vi "风速测量.vi"() -> ()   [LabVIEW 2014]
panel:
  in  "输入设备":tag="Dev2/port0/line0:2"
  in  "输出设备":tag="Dev1/port0/line0:7"
  out "测量点":u32[](array[numeric])
  out "Error Out":errorcluster caption="错误输出"
  in  "风筒直径":string
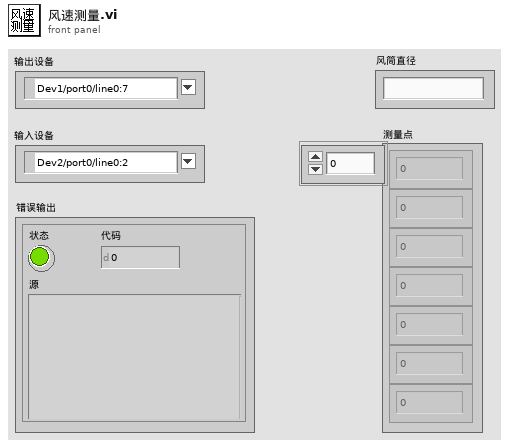
[diagram p1: front panel]
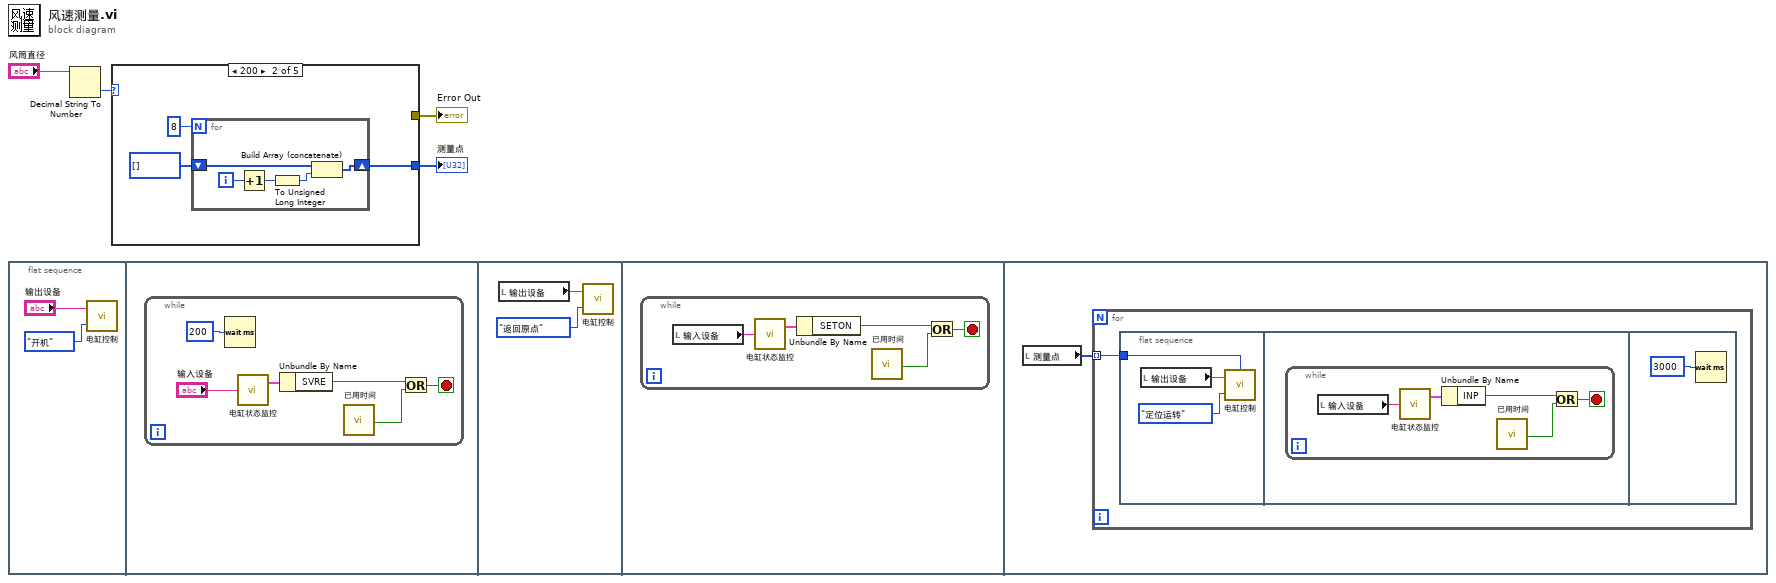
[diagram p0: block diagram]
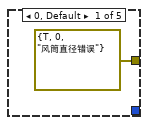
[diagram p2: hidden frame]
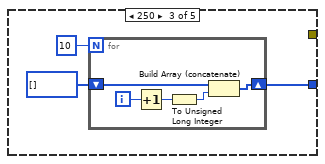
[diagram p3: hidden frame]
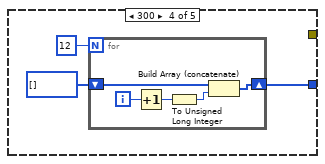
[diagram p4: hidden frame]
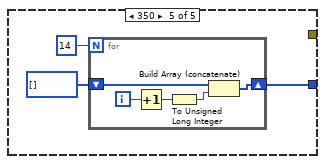
[diagram p5: hidden frame]
diagram:
  n1 = flat-sequence {
    frame #0 {
      n2 = call "电缸控制.vi"("枚举"=enum16{"开机", "返回原点", "定位运转", "报警复位"}."开机", "输出设备"="输出设备") -> ()  [unwired: 1 in, 1 out]
    }
    frame #1 {
      n3 = while {
        stop <- w9 stop-if-true
        n4 = Wait (ms)(milliseconds to wait=u32 200 ("等待时间（毫秒）")) -> ()  [unwired: 1 out]
        n5 = call "电缸状态监控.vi"("输入设备"="输入设备") -> ("电缸状态指示"=w12:cluster{"INP":bool, "SETON":bool, "SVRE":bool})  [unwired: 1 out]
        n6 = Unbundle By Name(w12) -> ("SVRE"=w11:bool)
        n7 = call "已用时间"() -> ("Time has Elapsed"=w10:bool)  [unwired: 12 in, 7 out]
        n8 = Or(x=w11, y=w10) -> (x .or. y?=w9:bool)
      }
    }
    frame #2 {
      n9 = local read "输出设备"() -> (w14:tag)
      n10 = call "电缸控制.vi"("枚举"=enum16{"开机", "返回原点", "定位运转", "报警复位"}."返回原点", "输出设备"=w14) -> ()  [unwired: 1 in, 1 out]
    }
    frame #3 {
      n11 = while {
        stop <- w15 stop-if-true
        n12 = local read "输入设备"() -> (w16:tag)
        n13 = call "电缸状态监控.vi"("输入设备"=w16) -> ("电缸状态指示"=w19:cluster{"INP":bool, "SETON":bool, "SVRE":bool})  [unwired: 1 out]
        n14 = Unbundle By Name(w19) -> ("SETON"=w18:bool)
        n15 = call "已用时间"() -> ("Time has Elapsed"=w17:bool)  [unwired: 12 in, 7 out]
        n16 = Or(x=w18, y=w17) -> (x .or. y?=w15:bool)
      }
    }
    frame #4 {
      n17 = local read "测量点"() -> (w20:u32[])
      n18 = for {
        tunnel: w20 -> [w21] mode=indexing
        n19 = flat-sequence {
          tunnel: w21 -> [w22]
          frame #0 {
            n20 = local read "输出设备"() -> (w23:tag)
            n21 = call "电缸控制.vi"("步序号"=w22, "枚举"=enum16{"开机", "返回原点", "定位运转", "报警复位"}."定位运转", "输出设备"=w23) -> ()  [unwired: 1 out]
          }
          frame #1 {
            n22 = while {
              stop <- w25 stop-if-true
              n23 = local read "输入设备"() -> (w26:tag)
              n24 = call "电缸状态监控.vi"("输入设备"=w26) -> ("电缸状态指示"=w29:cluster{"INP":bool, "SETON":bool, "SVRE":bool})  [unwired: 1 out]
              n25 = Unbundle By Name(w29) -> ("INP"=w28:bool)
              n26 = call "已用时间"() -> ("Time has Elapsed"=w27:bool)  [unwired: 12 in, 7 out]
              n27 = Or(x=w28, y=w27) -> (x .or. y?=w25:bool)
            }
          }
          frame #2 {
            n28 = Wait (ms)(milliseconds to wait=u32 3000 ("等待时间（毫秒）")) -> ()  [unwired: 1 out]
          }
        }
      }
    }
  }
  n29 = Decimal String To Number(string="风筒直径") -> (number=w3:i32)  [unwired: 2 in, 1 out]
  n30 = case shown="200" w3 {
    tunnel: [errorcluster {"status"=TRUE, "code"=0, "source"="风筒直径错误"} ("Error Out") _ _ _ _] -> w1
    tunnel: [_ w34 w40 w48 w56] -> w2
    frame 0, Default {
    }
    frame 200 {
      n31 = for {
        N: 8 -> [_]
        shift-right: [w37] -> w34
        shift-left: u32[] [] -> [w39]
        i -> [w35]
        n32 = Increment(x=w35) -> (x+1=w36:i32)
        n33 = To Unsigned Long Integer(number=w36) -> (unsigned 32bit integer=w38:u32)
        n34 = Build Array (concatenate)(w39, w38) -> (w37:u32[])
      }
    }
    frame 250 {
      n35 = for {
        N: 10 -> [_]
        shift-right: [w45] -> w40
        shift-left: u32[] [] -> [w47]
        i -> [w44]
        n36 = Increment(x=w44) -> (x+1=w43:i32)
        n37 = To Unsigned Long Integer(number=w43) -> (unsigned 32bit integer=w46:u32)
        n38 = Build Array (concatenate)(w47, w46) -> (w45:u32[])
      }
    }
    frame 300 {
      n39 = for {
        N: 12 -> [_]
        shift-right: [w53] -> w48
        shift-left: u32[] [] -> [w55]
        i -> [w52]
        n40 = Increment(x=w52) -> (x+1=w51:i32)
        n41 = To Unsigned Long Integer(number=w51) -> (unsigned 32bit integer=w54:u32)
        n42 = Build Array (concatenate)(w55, w54) -> (w53:u32[])
      }
    }
    frame 350 {
      n43 = for {
        N: 14 -> [_]
        shift-right: [w61] -> w56
        shift-left: u32[] [] -> [w63]
        i -> [w60]
        n44 = Increment(x=w60) -> (x+1=w59:i32)
        n45 = To Unsigned Long Integer(number=w59) -> (unsigned 32bit integer=w62:u32)
        n46 = Build Array (concatenate)(w63, w62) -> (w61:u32[])
      }
    }
  }
  "Error Out" <- w1
  "测量点" <- w2
